vi "generate header file.vi"(7 "engine in":refnum<class "Engine Parent Editor Node.lvclass">, 8 "error in (no error)":errorcluster, 9 "write to file? (T)":bool=TRUE, 10 "file path":path, 11 "shared memory editor node in":refnum<class "module editor node.lvclass">) -> (0 "error out":errorcluster, 2 "generation output":string, 3 "shared memory editor node out":refnum<class "module editor node.lvclass">, 5 "engine out":refnum<class "Engine Parent Editor Node.lvclass">)   [LabVIEW 2014, in "Shared Memory editor node.lvclass"]
uses:
  Shared Memory editor node.lvclass
  <vilib>/NI/DCAF/Tag Editor Core/Configuration Editor/Classes/Module editor node/module editor node.lvclass
  <vilib>/NI/DCAF/Tag Editor Core/Configuration Editor/Classes/Engine Parent/Engine Parent Editor Node.lvclass
  cheddar/C Header Generator.lvlib
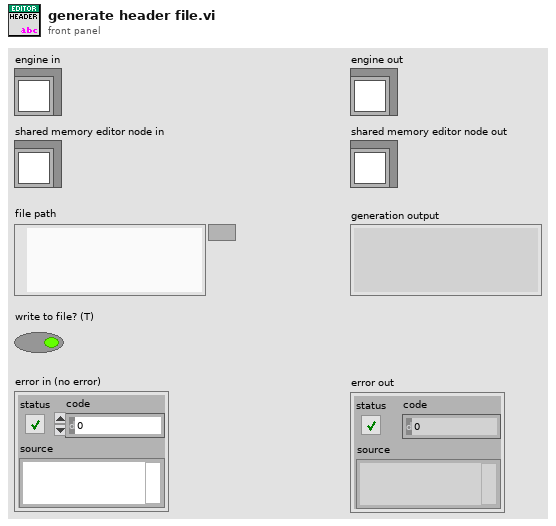
[diagram p1: front panel]
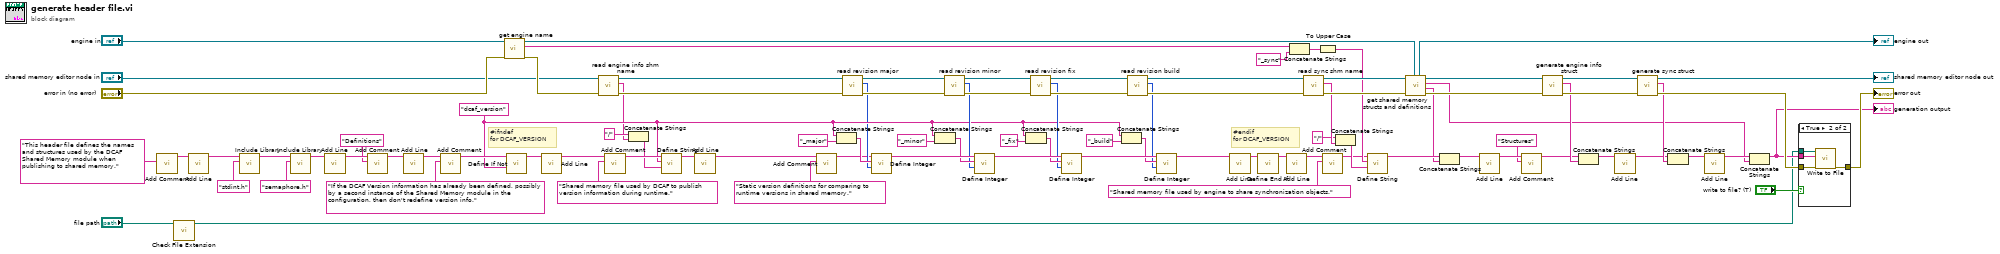
[diagram p0: block diagram]
diagram:
  w16 = "dcaf_version" ("token string")
  # "#ifndef\nfor DCAF_VERSION"
  # "#endif\nfor DCAF_VERSION"
  n1 = call "Add Comment.vi"("Comment"="This header file defines the names and structures used by the DCAF Shared Memory module when publishing to shared memory.") -> ("String out"=w92:string)  [unwired: 10 in]
  n2 = call "Check File Extension.vi"("path in"="file path") -> ("path out"=w45:path)  [unwired: 10 in]
  n3 = call "Add Line.vi"("String in"=w92) -> ("String out"=w53:string)  [unwired: 10 in]
  n4 = call "Include Library.vi"("Library Name"="stdint.h", "String in"=w53) -> ("String out"=w52:string)  [unwired: 9 in]
  n5 = call "Include Library.vi"("Library Name"="semaphore.h", "String in"=w52) -> ("String out"=w51:string)  [unwired: 9 in]
  n6 = call "Add Line.vi"("String in"=w51) -> ("String out"=w50:string)  [unwired: 10 in]
  n7 = call "Add Comment.vi"("Comment"="Definitions", "String in"=w50) -> ("String out"=w22:string)  [unwired: 9 in]
  n8 = call "Add Line.vi"("String in"=w22) -> ("String out"=w21:string)  [unwired: 10 in]
  n9 = call "Add Comment.vi"("Comment"="If the DCAF Version information has already been defined, possibly by a second instance of the Shared Memory module in the configuration, then don't redefine version info.", "String in"=w21) -> ("String out"=w35:string)  [unwired: 9 in]
  n10 = call "get engine name.vi"("error in (no error)"="error in (no error)", "engine in"="engine in") -> ("error out"=w14:errorcluster, "engine name"=w36:string, "engine out"=w72:refnum<class "Engine Parent Editor Node.lvclass">)  [unwired: 7 in]
  n11 = call "Define If Not.vi"("token string"=w16, "String in"=w35) -> ("String out"=w28:string)  [unwired: 9 in]
  n12 = call "Add Line.vi"("String in"=w28) -> ("String out"=w18:string)  [unwired: 10 in]
  n13 = call "read engine info shm name.vi"("error in"=w14, "shared memory editor node"="shared memory editor node in") -> ("error out"=w13:errorcluster, "shm name"=w11:string, "shared memory editor node out"=w12:refnum<class "module editor node.lvclass">)  [unwired: 7 in]
  n14 = call "Add Comment.vi"("Comment"="Shared memory file used by DCAF to publish version information during runtime.", "String in"=w18) -> ("String out"=w17:string)  [unwired: 9 in]
  n15 = Concatenate Strings("/" ("string"), w11) -> (w15:string)
  n16 = call "Define String.vi"("Value"=w15, "Name"=w16, "String in"=w17) -> ("String out"=w9:string)  [unwired: 8 in]
  n17 = call "Add Line.vi"("String in"=w9) -> ("String out"=w7:string)  [unwired: 10 in]
  n18 = call "Add Comment.vi"("Comment"="Static version definitions for comparing to runtime versions in shared memory.", "String in"=w7) -> ("String out"=w6:string)  [unwired: 9 in]
  n19 = Concatenate Strings(w16, "_major" ("string")) -> (w34:string)
  n20 = call "read revision major.vi"("error in"=w13, "shared memory editor node"=w12) -> ("error out"=w86:errorcluster, "revision major"=w8:u16, "shared memory editor node out"=w85:refnum<class "module editor node.lvclass">)  [unwired: 7 in]
  n21 = call "Define Integer.vi"("Value"=w8, "Name"=w34, "String in"=w6) -> ("String out"=w84:string)  [unwired: 8 in]
  n22 = Concatenate Strings(w16, "_minor" ("string")) -> (w33:string)
  n23 = call "read revision minor.vi"("error in"=w86, "shared memory editor node"=w85) -> ("error out"=w40:errorcluster, "revision minor"=w30:u16, "shared memory editor node out"=w38:refnum<class "module editor node.lvclass">)  [unwired: 7 in]
  n24 = call "Define Integer.vi"("Value"=w30, "Name"=w33, "String in"=w84) -> ("String out"=w41:string)  [unwired: 8 in]
  n25 = Concatenate Strings(w16, "_fix" ("string")) -> (w32:string)
  n26 = call "read revision fix.vi"("error in"=w40, "shared memory editor node"=w38) -> ("error out"=w39:errorcluster, "revision fix"=w29:u16, "shared memory editor node out"=w37:refnum<class "module editor node.lvclass">)  [unwired: 7 in]
  n27 = call "Define Integer.vi"("Value"=w29, "Name"=w32, "String in"=w41) -> ("String out"=w42:string)  [unwired: 8 in]
  n28 = Concatenate Strings(w16, "_build" ("string")) -> (w31:string)
  n29 = call "read revision build.vi"("error in"=w39, "shared memory editor node"=w37) -> ("error out"=w4:errorcluster, "revision build"=w3:u16, "shared memory editor node out"=w2:refnum<class "module editor node.lvclass">)  [unwired: 7 in]
  n30 = call "Define Integer.vi"("Value"=w3, "Name"=w31, "String in"=w42) -> ("String out"=w5:string)  [unwired: 8 in]
  n31 = call "Add Line.vi"("String in"=w5) -> ("String out"=w26:string)  [unwired: 10 in]
  n32 = call "Define End If.vi"("String in"=w26) -> ("String out"=w27:string)  [unwired: 10 in]
  n33 = call "Add Line.vi"("String in"=w27) -> ("String out"=w25:string)  [unwired: 10 in]
  n34 = Concatenate Strings(w36, "_sync" ("Name")) -> (w70:string)
  n35 = call "read sync shm name.vi"("error in"=w4, "shared memory editor node"=w2) -> ("error out"=w79:errorcluster, "shm name"=w78:string, "shared memory editor node out"=w80:refnum<class "module editor node.lvclass">)  [unwired: 7 in]
  n36 = To Upper Case(1:w70) -> (0:w69:string)
  n37 = call "Add Comment.vi"("Comment"="Shared memory file used by engine to share synchronization objects.", "String in"=w25) -> ("String out"=w24:string)  [unwired: 9 in]
  n38 = Concatenate Strings("/" ("string"), w78) -> (w77:string)
  n39 = call "Define String.vi"("Value"=w77, "Name"=w69, "String in"=w24) -> ("String out"=w60:string)  [unwired: 8 in]
  n40 = call "get shared memory structs and definitions.vi"("engine in"=w72, "error in (no error)"=w79, "editor node in"=w80) -> ("error out"=w95:errorcluster, "shm file definitions"=w58:string, "shm data structs"=w56:string, "editor node out"=w67:refnum<class "module editor node.lvclass">, "engine out"=→"engine out":refnum<class "Engine Parent Editor Node.lvclass">)  [unwired: 4 in]
  n41 = Concatenate Strings(w60, w58) -> (w59:string)
  n42 = call "Add Line.vi"("String in"=w59) -> ("String out"=w91:string)  [unwired: 10 in]
  n43 = call "Add Comment.vi"("Comment"="Structures", "String in"=w91) -> ("String out"=w62:string)  [unwired: 9 in]
  n44 = call "generate engine info struct.vi"("error in (no error)"=w95, "shared memory editor node in"=w67) -> ("error out"=w65:errorcluster, "struct string"=w63:string, "shared memory editor node out"=w66:refnum<class "module editor node.lvclass">)  [unwired: 7 in]
  n45 = Concatenate Strings(w62, w63) -> (w64:string)
  n46 = call "Add Line.vi"("String in"=w64) -> ("String out"=w61:string)  [unwired: 10 in]
  n47 = call "generate sync struct.vi"("error in (no error)"=w65, "shared memory editor node in"=w66) -> ("error out"=w94:errorcluster, "struct string"=w88:string, "shared memory editor node out"=→"shared memory editor node out":refnum<class "module editor node.lvclass">)  [unwired: 7 in]
  n48 = Concatenate Strings(w61, w88) -> (w81:string)
  n49 = call "Add Line.vi"("String in"=w81) -> ("String out"=w57:string)  [unwired: 10 in]
  n50 = Concatenate Strings(w57, w56) -> (w47:string)
  "generation output" <- w47
  n51 = case shown="True" "write to file? (T)" {
    tunnel: w94 -> [w96 w100]
    tunnel: w45 -> [_ w99]
    tunnel: w47 -> [_ w98]
    tunnel: [w96 w97] -> w49
    frame False {
    }
    frame True {
      n52 = call "Write to File.vi"("error in (no error)"=w100, "header text"=w98, "file path"=w99) -> ("error out"=w97:errorcluster)  [unwired: 8 in]
    }
  }
  "error out" <- w49
